vi "[ex ce]_Array - Access 2D Array elements.vi"() -> ()   [LabVIEW 2021]
doc: "<B>Example for CalcExpress script syntax</B>\n\n<B>The VI demonstrates various methods of accessing elements in 2D array</B>\n\nThis example demonstrates a use of Index Arrays and Index Ranges to perform array indexing. IndexRange feature lets you specify a sequential index subset of an array dimension. Index Array can be used to specify an arbitrary set of indeces.\n\nTo provide the Index Range feature, CalcExpress supports IndexRange Operator, IndexRange Symbols and a few IndexRange Functions. Despite they have different syntax, they have the similar functionality, so you can use any of them to specify range of indeces. In general, IndexRange symbols and functions can be convenient if you need to specify entire dimension, and IndexRange Operator can be convenient if you need to specify a sequential index subset.\n\n::: CalcExpress Toolkit :::\nCopyright (c) 2000-2026 Konstantin Shifershteyn. All rights reserved."
panel:
  in  "stop":bool
  in  "calc":bool
  in  "Expression":string
  in  "comments":string="This example demonstrates a use of Index Arrays and Index Ranges to perform array indexing. IndexRange feature lets you specify a sequential index subset of an array dimension. Index Array can be used to specify an arbitrary set of indeces.\n\nTo provide the Index Range feature, CalcExpress supports IndexRange Operator, IndexRange Symbols and a few IndexRange Functions. Despite they have different syntax, they have the similar functionality, so you can use any of them to specify range of indeces.  In general, IndexRange symbols and functions can be convenient if you need to specify entire dimension, and IndexRange Operator can be convenient if you need to specify a sequential index subset.\n"
  in  "Expressions":string[](array[string])=["iRow = 1;  //row index\n\nrow  = x[iRow];\n/*  Row value. It is similar to:\nrow = x[iRow, $>];\nrow = x[iRow, 0:cols(x)];\n*/\n\nrowr = x[iRow, $<];\n/*  Reversed Row value. It's similar to:\nrowr = x[iRow, cols(x):0]; \n*/\n\nsubr = x[iRow, 1:3];\n/* Subset of row (columns 1,2,3) */\n\n/* Show results */\nprobe(row,  \"Row value\");\nprobe(rowr, \"Reversed Row\");\nprobe(subr, \"Row subset\");\n", "iCol = 1;  //column index\n\ncol  = x[$>, iCol];\n/*  Column value. It is similar to:\ncol = x[0:rows(x), iCol];\n*/\n\ncolr = x[$<, iCol];\n/*  Reversed column value. It's similar to:\nrowr = x[rows(x):0, iCol]; \n*/\n\nsubc = x[1:3, iCol];\n/* Subset of column (rows 1,2,3) */\n\n/* Show results */\nprobe(col,  \"Column value\");\nprobe(colr, \"Reversed Column\");\nprobe(subc, \"Column subset\");\n", "mDiag = x[$> @ $>];\n/*  Main diagonal. It is similar to:\nmDiag = x[0:rows(x) @ 0:cols(x)];\n*/\n\ncDiag = x[$> @ $<];\n/*  Collateral diagonal. It's similar to:\ncDiag = x[0:rows(x) @ cols(x):0]; \n*/\n\nsDiag = x[1:3 @ 1:3];\n/* Subset of main diagonal */\n\n/* Show results */\nprobe(mDiag, \"Main Diagonal\");\nprobe(cDiag, \"Collateral Diagonal\");\nprobe(sDiag, \"Subset of main diagonal\");\n", "subsetA = x[1:2];\n/* Result is 2D array that consist of 1st and 2nd rows of x. Similar result can be obtained if you use\nsubsetA = x[1:2, 0:cols(x)]; or\nsubsetA = x[1:2, $>];\n*/\n\nsubsetB = x[$>, 3:2];\n/* Result is 2D array that consist of 3rd and 2nd columns of x (Pay attention to the order). Similar result can be obtained if you use\nsubsetB = x[0:rows(x), 3:2];\n*/\n\nsubsetC = x[1:3, 0:1];\n/* Result is 2D array that is intersection of rows from 1 to 3, and columns from 0 to 1 of x.\n*/\n\nprobe( subsetA, \"Subset A\");\nprobe( subsetB, \"Subset B\");\nprobe( subsetC, \"Subset C\");\n", "y1 = y2 = y3 = y4 = x;\n/* makes copies of x */\n\ny1[1] = -10;\n/* Fills a row. */ \n\ny2[2] = vector(-10,-20,-30,-40, -50);\n/* Assigns 1D array to row */\n\ny3[$>, 1] = nvecins(-100,rows(y3),-1);\n/* Assigns 1D array to column */\n\ny4[$> @ $>] = 1000;\n/* Fills the main diagonal */\n\nprobe( y1, \"y1\");\nprobe( y2, \"y2\");\nprobe( y3, \"y3\");\nprobe( y4, \"y4\");\n", "z1 = z2 = z3 = z4 = x;\n/* makes copies of x */\n\nz1[1:3, 0:1] = -100;\n/* Fills a subset */\n\nz2[1:3, 0:1] = vector(-800, -900);\n/* Assigns 1D array to subset */\n\nz3[1:3, 0:1] = nmtxins(-1000,5,-1);\n/* Assigns 2D array to subset */\n\nz4[$>, $>] = 0;\n/* Fills entire array. Also can be written as\nz4[0:rows(z4), 0:cols(z4)] = 0;\nNote, you can't use z4=0 because an assignment operator requires its operands have the same datatype */\n\nprobe(z1, \"z1\");\nprobe(z2, \"z2\");\nprobe(z3, \"z3\");\nprobe(z4, \"z4\");\n", "idx0 = vector(0,2,4);\nidx1 = vector(1,3,4);\n\ny = x[idx0,idx1];\n/*\n Result is 2D array that consists of elements of x located on intersection of rows 0,2,4 and columns 1,3,4\n*/\n\nprobe(y, \"y\");\n"]
  in  "sel":i32(ring) items=["Indexing rows", "Indexing columns", "Indexing diagonals", "Indexing 2D subsets", "Assigning rows, columns, and diagonals", "Assigning 2D subsets", "Using Index Array"]
  in  "x":dbl[][](array[numeric])=[[0.0, 0.1, 0.2, 0.3, 0.4], [1.0, 1.1, 1.2, 1.3, 1.4], [2.0, 2.1, 2.2, 2.3, 2.4], [3.0, 3.1, 3.2, 3.3, 3.4], [4.0, 4.1, 4.2, 4.3, 4.4]] caption="(source 2D array)" format="%.1f"
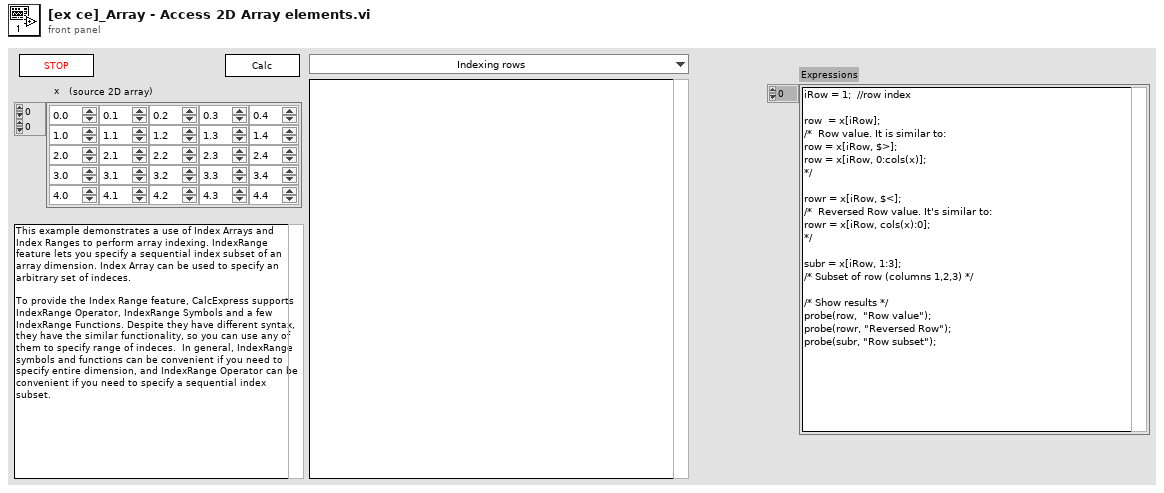
[diagram p1: front panel]
types:
  T1 = enum16{"create", "destroy", "set value", "get value"}
  T2 = typedef "VarMan Variable Context Handle.ctl" = i32
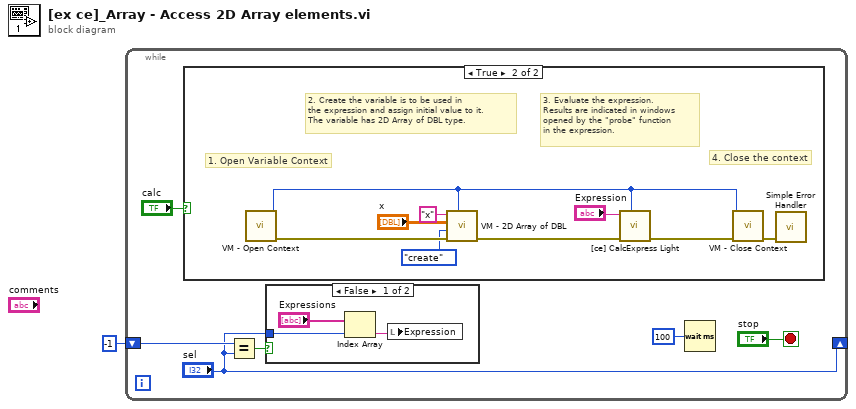
[diagram p0: block diagram]
diagram:
  n1 = while {
    shift-left: -1 ("sel") -> [w7]
    shift-right: ["sel"] -> _
    stop <- "stop" stop-if-true
    n2 = case shown="True" "calc" {
      frame False {
      }
      frame True {
        # "3. Evaluate the expression.\nResults are indicated in windows\nopened by the \"probe\" function\nin the expression."
        # "4. Close the context"
        # "2. Create the variable is to be used in\nthe expression and assign initial value to it.\nThe variable has 2D Array of DBL type."
        # "1. Open Variable Context"
        n3 = call "VM - Open Context.vi"() -> ("error out"=w19:errorcluster, "VC Handle out"=w13:T2)  [unwired: 9 in, 1 out]
        n4 = call "VM - 2D Array of DBL.vi"("VC Handle"=w13, "error in"=w19, "cmd"=T1."create", "value in"="x", "name_spec"="x" ("name")) -> ("error out"=w18:errorcluster)  [unwired: 1 in, 5 out]
        n5 = call "[ce] CalcExpress Light.vi"("VC Handle"=w13, "error in"=w18, "expression"="Expression") -> ("error out"=w12:errorcluster)  [unwired: 6 in, 2 out]
        n6 = call "VM - Close Context.vi"("error in"=w12, "VC Handle"=w13) -> ("error out"=w17:errorcluster)  [unwired: 8 in, 1 out]
        n7 = call <vilib>:"Simple Error Handler.vi"("error in (no error)"=w17) -> ()  [unwired: 4 in, 5 out]
      }
    }
    n8 = Equal?(x=w7, y="sel") -> (x = y?=w6:bool)
    n9 = case shown="False" w6 {
      tunnel: "sel" -> [w9 _]
      frame False {
        n10 = Index Array(array="Expressions", index=w9) -> (element=w8:string)
        n11 = local write "Expression"(w8) -> ()
      }
      frame True {
      }
    }
    n12 = Wait (ms)(milliseconds to wait=u32 100) -> ()  [unwired: 1 out]
  }
